vi "GOOP_CreateDefaultIniFile.vi"() -> (1 "NativeRead":path, 2 "NativeWrite":path)   [LabVIEW 2020]
uses:
  ClassProviders/Provider_EndevoGOOP300/EndevoProviderName.ctl
  ClassProviders/Provider_LvNativeClass/LvNativeProviderName.ctl
  ClassProviders/Provider_EndevoGOOP400/EndevoG4ProviderName.ctl
  <vilib>/Utility/config.llb/Write Key (String).vi
  <vilib>/Utility/config.llb/NI_LVConfig.lvlib
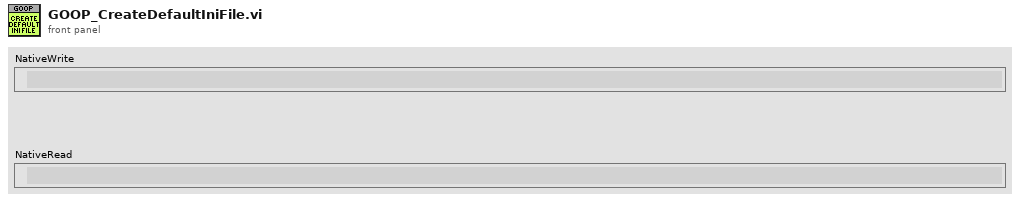
[diagram p1: front panel]
types:
  T1 = typedef "EndevoG4ProviderName.ctl" = enum16{"EndevoGOOP400"}
  T2 = typedef "LvNativeProviderName.ctl" = enum16{"Endevo LabVIEW Native"}
  T3 = typedef "EndevoProviderName.ctl" = enum16{"EndevoGOOP300"}
  T4 = typedef "NI_LVConfig.lvlib/Config Data RefNum.ctl" = refnum<k1>
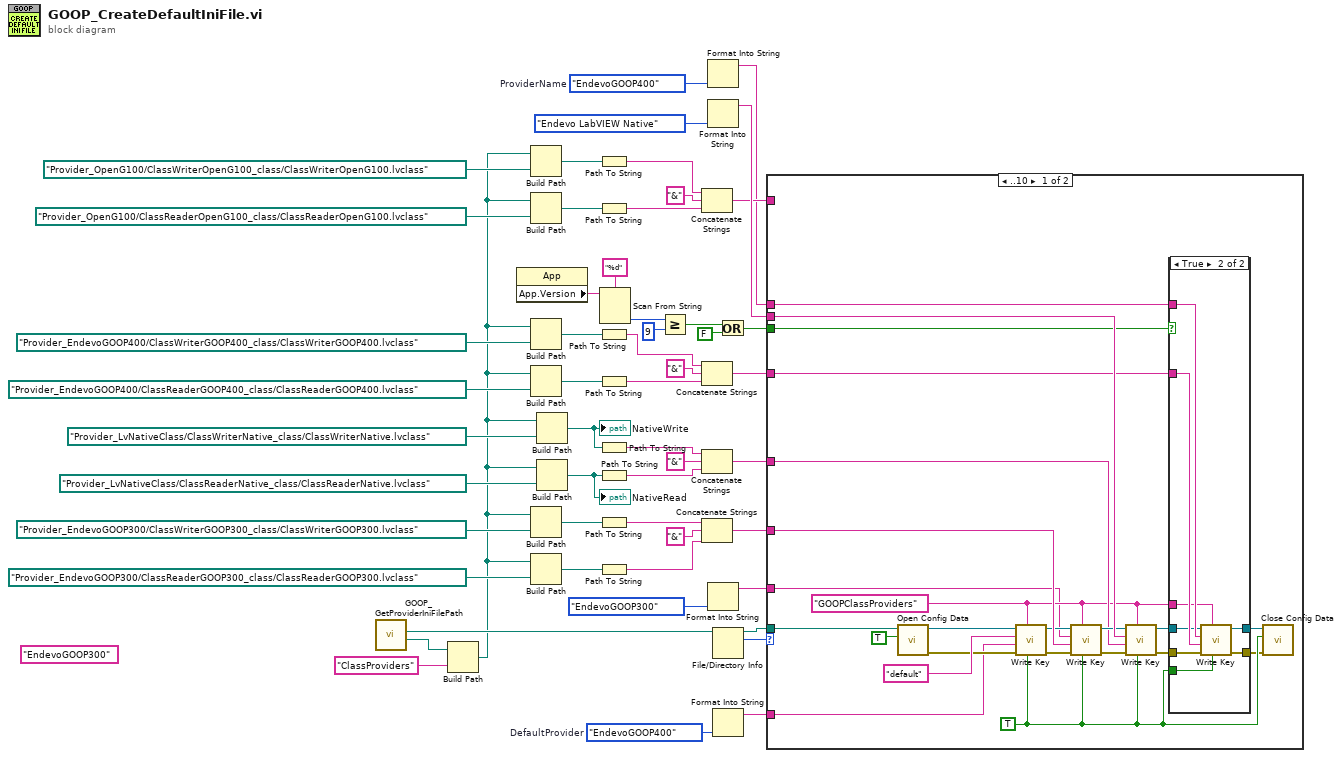
[diagram p0: block diagram]
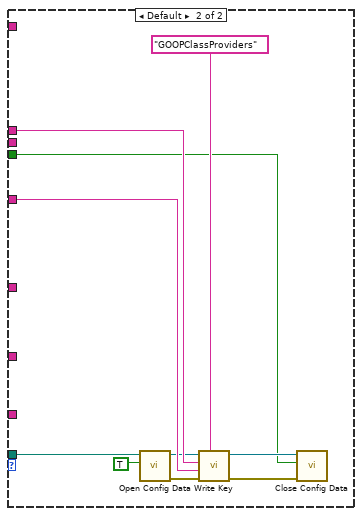
[diagram p3: hidden frame]
diagram:
  w2 = EndevoG4ProviderName."EndevoGOOP400"  # DefaultProvider
  w4 = EndevoG4ProviderName."EndevoGOOP400"  # ProviderName
  (unwired) "EndevoGOOP300" ("section")
  n1 = call "GOOP_GetProviderIniFilePath.vi"() -> ("ProviderMainFolder"=w22:path, "ProviderIniPath"=w50:path)  [unwired: 10 in]
  n2 = Build Path(base path=w22, name or relative path="ClassProviders") -> (appended path=w3:path)
  n3 = property class="App"() -> ("App.Version"=w16:string)  [unwired: 2 in, 2 out]
  n4 = Build Path(base path=w3, name or relative path=path "Provider_OpenG100/ClassWriterOpenG100_class/ClassWriterOpenG100.lvclass" ("base path")) -> (appended path=w30:path)
  n5 = Build Path(base path=w3, name or relative path=path "Provider_OpenG100/ClassReaderOpenG100_class/ClassReaderOpenG100.lvclass" ("base path")) -> (appended path=w29:path)
  n6 = Build Path(base path=w3, name or relative path=path "Provider_EndevoGOOP400/ClassWriterGOOP400_class/ClassWriterGOOP400.lvclass" ("base path")) -> (appended path=w8:path)
  n7 = Build Path(base path=w3, name or relative path=path "Provider_EndevoGOOP400/ClassReaderGOOP400_class/ClassReaderGOOP400.lvclass" ("base path")) -> (appended path=w9:path)
  n8 = Build Path(base path=w3, name or relative path=path "Provider_EndevoGOOP300/ClassWriterGOOP300_class/ClassWriterGOOP300.lvclass" ("base path")) -> (appended path=w37:path)
  n9 = Build Path(base path=w3, name or relative path=path "Provider_EndevoGOOP300/ClassReaderGOOP300_class/ClassReaderGOOP300.lvclass" ("base path")) -> (appended path=w36:path)
  n10 = Build Path(base path=w3, name or relative path=path "Provider_LvNativeClass/ClassWriterNative_class/ClassWriterNative.lvclass" ("base path")) -> (appended path=w31:path)
  "NativeWrite" <- w31
  n11 = Build Path(base path=w3, name or relative path=path "Provider_LvNativeClass/ClassReaderNative_class/ClassReaderNative.lvclass" ("base path")) -> (appended path=w23:path)
  "NativeRead" <- w23
  n12 = Path To String(path=w30) -> (string=w26:string)
  n13 = Path To String(path=w29) -> (string=w27:string)
  n14 = Path To String(path=w8) -> (string=w12:string)
  n15 = Path To String(path=w9) -> (string=w11:string)
  n16 = Path To String(path=w31) -> (string=w35:string)
  n17 = Path To String(path=w23) -> (string=w34:string)
  n18 = Path To String(path=w37) -> (string=w38:string)
  n19 = Path To String(path=w36) -> (string=w39:string)
  n20 = Scan From String(format string="%d", input string=w16) -> (output 1=w14:i32)  [unwired: 3 in, 3 out]
  n21 = Greater Or Equal?(x=w14, y=9) -> (x >= y?=w7:bool)
  n22 = Concatenate Strings(w26, "&" ("regular expression"), w27) -> (w25:string)
  n23 = Concatenate Strings(w12, "&" ("regular expression"), w11) -> (w20:string)
  n24 = Concatenate Strings(w35, "&" ("regular expression"), w34) -> (w32:string)
  n25 = Concatenate Strings(w38, "&" ("regular expression"), w39) -> (w41:string)
  n26 = Format Into String(w4) -> (resulting string=w17:string)  [unwired: 3 in, 1 out]
  n27 = Format Into String(LvNativeProviderName."Endevo LabVIEW Native" ("ProviderName")) -> (resulting string=w42:string)  [unwired: 3 in, 1 out]
  n28 = Format Into String(EndevoProviderName."EndevoGOOP300" ("ProviderName")) -> (resulting string=w51:string)  [unwired: 3 in, 1 out]
  n29 = File/Directory Info(path=w50) -> (path out=w53:path, size=w24:i64)  [unwired: 1 in, 5 out]
  n30 = Format Into String(w2) -> (resulting string=w1:string)  [unwired: 3 in, 1 out]
  n31 = Or(x=w7, y=FALSE) -> (x .or. y?=w6:bool)
  n32 = case shown="..10" w24 {
    tunnel: w53 -> [w76 w96]
    tunnel: w51 -> [w54 _]
    tunnel: w42 -> [w75 _]
    tunnel: w41 -> [w70 _]
    tunnel: w32 -> [w65 _]
    tunnel: w25 -> [_ _]
    tunnel: w17 -> [w63 w93]
    tunnel: w20 -> [w64 w94]
    tunnel: w6 -> [w58 w87]
    tunnel: w1 -> [w55 _]
    frame ..10 {
      w59 = TRUE ("write configuration file? (T)")
      w60 = "GOOPClassProviders" ("section")
      n33 = call <vilib>:"Open Config Data.vi"("create file if necessary (T)"=TRUE ("create file if necessary? (T)"), "configuration file path"=w76) -> ("error out"=w72:errorcluster, "refnum"=w71:T4)  [unwired: 7 in, 1 out]
      n34 = call-poly <vilib>:"Write Key.vi"("write raw string? (F)"=w59, "section"=w60, "error in (no error)"=w72, "value"=w55, "key"="default", "refnum"=w71) -> ("error out"=w69:errorcluster, "refnum out"=w68:T4)  [unwired: 3 in, 1 out]
      n35 = call-poly <vilib>:"Write Key.vi"("write raw string? (F)"=w59, "section"=w60, "error in (no error)"=w69, "value"=w70, "key"=w54, "refnum"=w68) -> ("error out"=w67:errorcluster, "refnum out"=w66:T4)  [unwired: 3 in, 1 out]
      n36 = call-poly <vilib>:"Write Key.vi"("write raw string? (F)"=w59, "section"=w60, "error in (no error)"=w67, "value"=w65, "key"=w75, "refnum"=w66) -> ("error out"=w61:errorcluster, "refnum out"=w62:T4)  [unwired: 3 in, 1 out]
      n37 = case shown="True" w58 {
        tunnel: w64 -> [_ w86]
        tunnel: w63 -> [_ w85]
        tunnel: w62 -> [w78 w84]
        tunnel: w61 -> [w77 w83]
        tunnel: [w77 w82] -> w57
        tunnel: [w78 w81] -> w56
        tunnel: w60 -> [_ w80]
        tunnel: w59 -> [_ w79]
        frame False {
        }
        frame True {
          n38 = call-poly <vilib>:"Write Key.vi"("write raw string? (F)"=w79, "section"=w80, "error in (no error)"=w83, "value"=w86, "key"=w85, "refnum"=w84) -> ("error out"=w82:errorcluster, "refnum out"=w81:T4)  [unwired: 3 in, 1 out]
        }
      }
      n39 = call <vilib>:"Close Config Data.vi"("error in (no error)"=w57, "write file if changed (T)"=w59, "refnum"=w56) -> ()  [unwired: 7 in, 2 out]
    }
    frame Default {
      n40 = call <vilib>:"Open Config Data.vi"("create file if necessary (T)"=TRUE ("create file if necessary? (T)"), "configuration file path"=w96) -> ("error out"=w90:errorcluster, "refnum"=w91:T4)  [unwired: 7 in, 1 out]
      n41 = call-poly <vilib>:"Write Key.vi"("section"="GOOPClassProviders", "error in (no error)"=w90, "value"=w94, "key"=w93, "refnum"=w91) -> ("error out"=w88:errorcluster, "refnum out"=w89:T4)  [unwired: 4 in, 1 out]
      n42 = call <vilib>:"Close Config Data.vi"("error in (no error)"=w88, "write file if changed (T)"=w87, "refnum"=w89) -> ()  [unwired: 7 in, 2 out]
    }
  }
